vi "Close.vi"(8 "error in (no error)":errorcluster, 11 "ToastFromXML in":refnum<class "ToastFromXML.lvclass">) -> (0 "error out":errorcluster)   [LabVIEW 2026, in "ToastNotification.lvlib" / "ToastFromXML.lvclass"]
doc: "Release the XML Document owned by this ToastFromXML source. Executes even on incoming error and merges the incoming error before release errors. No source output is returned. Class copies share the reference and must no longer use it after Close. Does not unregister service callbacks or dismiss the Windows notification."
uses:
  ToastFromXML.lvclass
  ToastFromXML.lvclass/ToastFromXML.ctl
  Read XML Document.vi
  Reflection DotNet/Reflection DotNet.lvlib
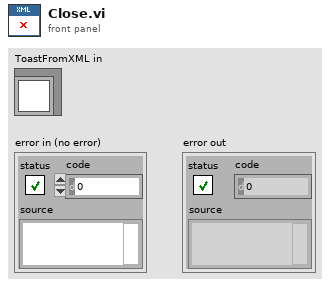
[diagram p1: front panel]
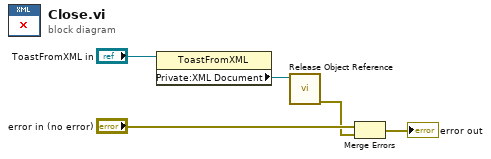
[diagram p0: block diagram]
diagram:
  n1 = property class="ToastFromXML"(reference="ToastFromXML in") -> ("Private:XML Document"=w2:refnum<k24>)  [unwired: 1 in, 2 out]
  n2 = call "Release Object Reference.vi"("object"=w2) -> ("error out"=w1:errorcluster)  [unwired: 10 in]
  n3 = Merge Errors("error in (no error)", w1) -> (→"error out":errorcluster)
